vi "Analog Irigation System.vi"() -> ()   [LabVIEW 2026]
panel:
  in  "Temperature Threshold":dbl
  in  "Temperature  Sensor :":dbl(slide) scale=0.0..30.0
  out "Mist Creator":bool
  out "Fan":bool
  out "Meter 2":dbl(knob) caption="Humidity  Indicator" scale=0.012..12.0
  in  "Sensitivity Potentiometer :":dbl(slide) scale=0.0..10.0
  in  "Humidity Sensor :":dbl(slide) scale=0.0..100.0
  out "Rain Lockout":bool
  out "Meter":dbl(knob) caption="Resistance  Indicator" scale=0.012..12.0
  in  "Vcc":dbl
  out "Tank  Empty/ Fault":bool
  in  "Flow & Current Sensor":bool
  in  "Tank Level Sensor":bool
  in  "Rain Lockout":bool
  in  "Sensitivity Potentiometer (Vref):":dbl(slide) scale=6.0..12.0
  in  "Soil Moisture Resistance (ohm):":dbl(slide) scale=1000.0..200000.0
  in  "?":bool
  in  "?":bool
  in  "?":bool
  out "Pump Running":bool
  out "Dry Soil":bool
  out "Power":bool
  # "Wet"
  # "Dry"
  # "Arid"
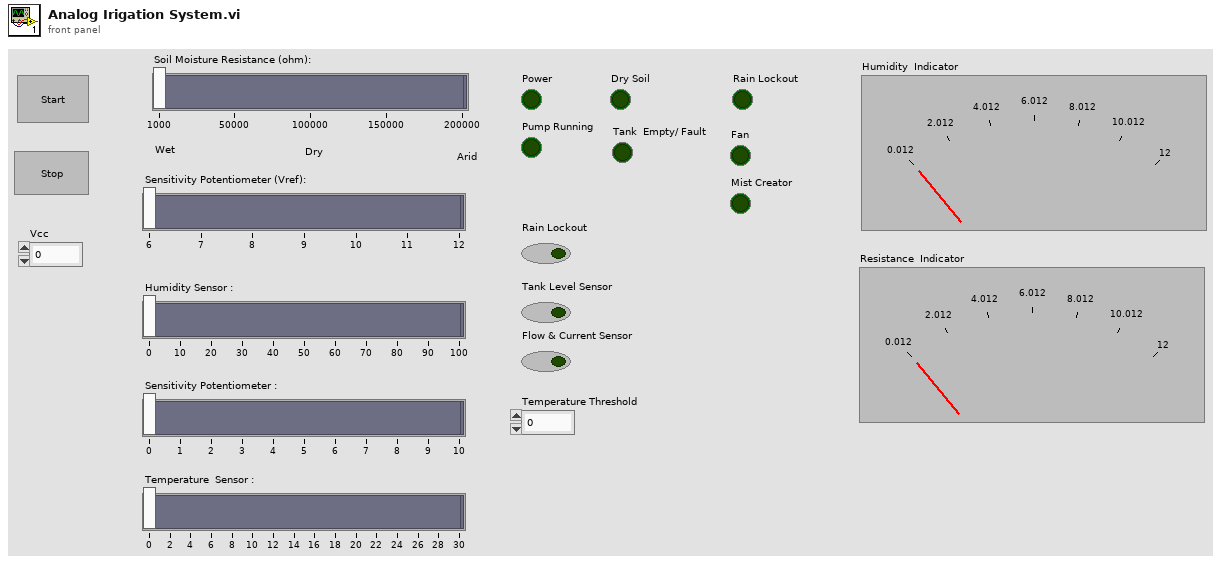
[diagram p1: front panel]
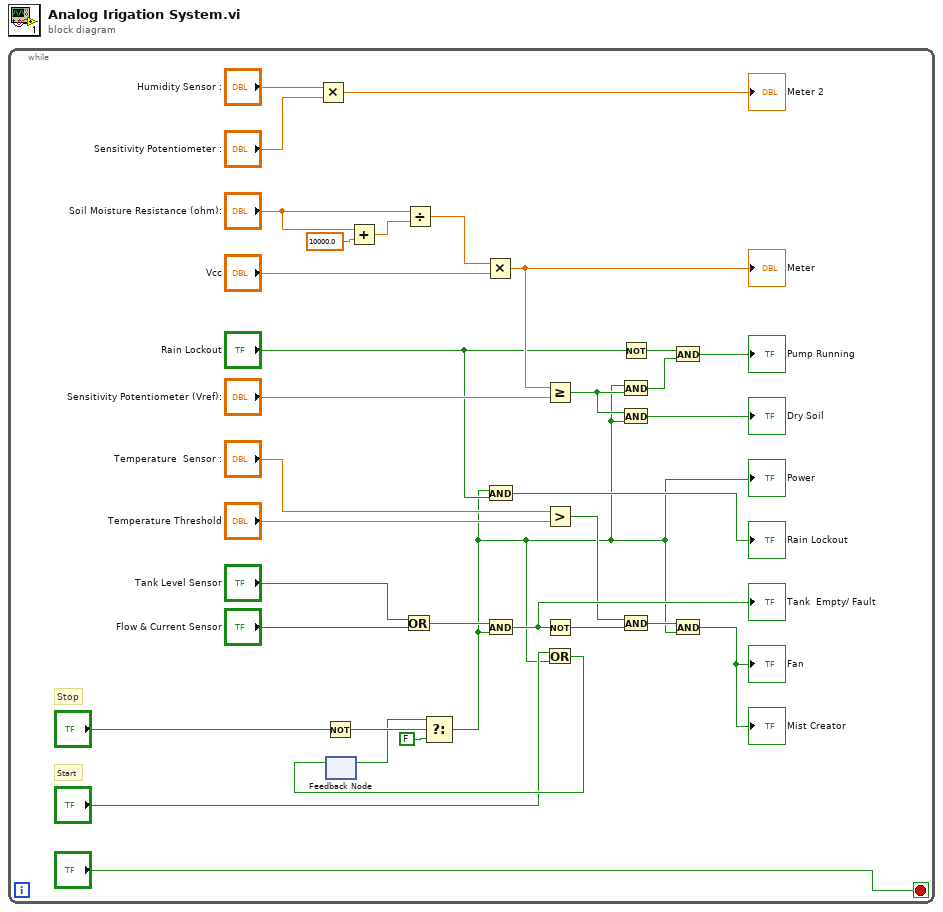
[diagram p0: block diagram]
diagram:
  n1 = while {
    stop <- "?" stop-if-true
    # "Stop"
    # "Start"
    n2 = Multiply(x="Humidity Sensor :", y="Sensitivity Potentiometer :") -> (x*y=→"Meter 2":dbl)
    n3 = Not(x="?") -> (.not. x?=w34:bool)
    n4 = feedback #1() -> (w31:bool)  [unwired: 1 in]
    n5 = Add(x="Soil Moisture Resistance (ohm):", y=10000.0) -> (x+y=w23:dbl)
    n6 = Or(x="Tank Level Sensor", y="Flow & Current Sensor") -> (x .or. y?=w26:bool)
    n7 = Divide(x="Soil Moisture Resistance (ohm):", y=w23) -> (x/y=w22:dbl)
    n8 = Select(t=w31, s=w34, f=FALSE) -> (s? t:f=w2:bool)
    "Power" <- w2
    n9 = Multiply(x=w22, y="Vcc") -> (x*y=w19:dbl)
    "Meter" <- w19
    n10 = And(x=w2, y="Rain Lockout") -> (x .and. y?=→"Rain Lockout":bool)
    n11 = And(x=w26, y=w2) -> (x .and. y?=w6:bool)
    "Tank  Empty/ Fault" <- w6
    n12 = Greater Or Equal?(x=w19, y="Sensitivity Potentiometer (Vref):") -> (x >= y?=w18:bool)
    n13 = Greater?(x="Temperature  Sensor :", y="Temperature Threshold") -> (0:w5:bool)
    n14 = Not(x=w6) -> (.not. x?=w4:bool)
    n15 = Or(x="?", y=w2) -> (x .or. y?=w35:bool)
    n16 = feedback-in #1(w35) -> ()
    n17 = Not(x="Rain Lockout") -> (.not. x?=w13:bool)
    n18 = And(x=w2, y=w18) -> (x .and. y?=w12:bool)
    n19 = And(x=w18, y=w2) -> (x .and. y?=→"Dry Soil":bool)
    n20 = And(x=w5, y=w4) -> (x .and. y?=w3:bool)
    n21 = And(x=w13, y=w12) -> (x .and. y?=→"Pump Running":bool)
    n22 = And(x=w3, y=w2) -> (x .and. y?=→"Fan" →"Mist Creator":bool)
  }
